vi "GetTestFilterv3.vi"() -> ()   [LabVIEW 2017]
uses:
  <vilib>/httpClient/LabVIEWHTTPClient.lvlib
panel:
  out "result string":string
  out "data":T1
  out "error out":errorcluster
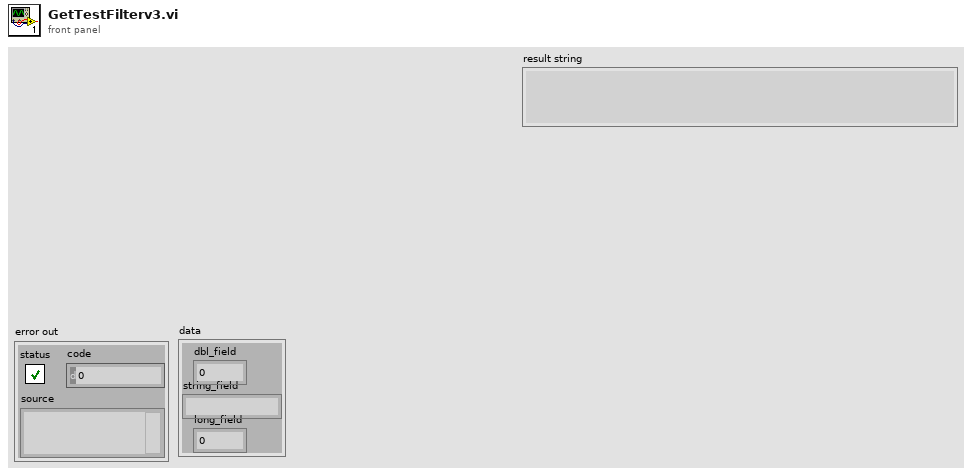
[diagram p1: front panel]
types:
  T1 = cluster{"dbl_field":dbl, "string_field":string, "long_field":i64}
  T2 = typedef "LabVIEWHTTPClient.lvlib/ClientHandle.ctl" = refnum<k1>
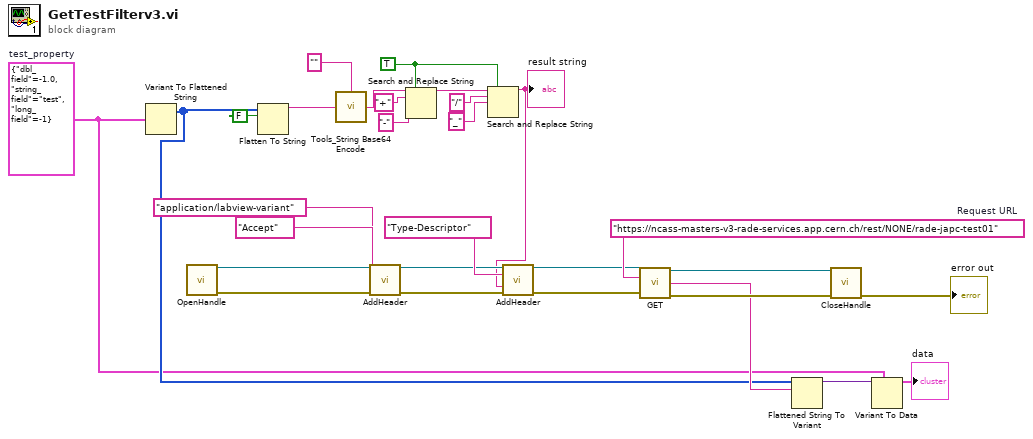
[diagram p0: block diagram]
diagram:
  w1 = T1 {"dbl_field"=-1.0, "string_field"="test", "long_field"=-1}  # test_property
  w7 = TRUE ("replace all? (F)")
  w26 = "https://ncass-masters-v3-rade-services.app.cern.ch/rest/NONE/rade-japc-test01"  # Request URL
  n1 = Variant To Flattened String(Variant=w1) -> (1:w2:i16[])  [unwired: 1 out]
  n2 = call <vilib>:"OpenHandle.vi"() -> ("client handle out"=w20:T2, "error out"=w19:errorcluster)  [unwired: 14 in]
  n3 = Flatten To String(anything=w2, prepend array or string size? (T)=FALSE) -> (data string=w13:string)  [unwired: 2 in, 2 out]
  n4 = call <userlib>:"Tools_String Base64 Encode.vi"("Normal String"=w13, "Line separator (\\n)"="") -> ("Base64 String"=w9:string)
  n5 = call <vilib>:"AddHeader.vi"("client handle"=w20, "header"="Accept", "value"="application/labview-variant", "error in (no error)"=w19) -> ("client handle out"=w18:T2, "error out"=w17:errorcluster)  [unwired: 10 in]
  n6 = Search and Replace String(replace all?=w7, input string=w9, search string="+" ("substring (\"\")"), replace string="-" ("replace string (\"\")")) -> (result string=w8:string)  [unwired: 4 in, 3 out]
  n7 = Search and Replace String(replace all?=w7, input string=w8, search string="/" ("substring (\"\")"), replace string="_" ("replace string (\"\")")) -> (result string=w3:string)  [unwired: 4 in, 3 out]
  "result string" <- w3
  n8 = call <vilib>:"AddHeader.vi"("client handle"=w18, "header"="Type-Descriptor", "value"=w3, "error in (no error)"=w17) -> ("client handle out"=w16:T2, "error out"=w15:errorcluster)  [unwired: 10 in]
  n9 = call <vilib>:"GET.vi"("client handle"=w16, "url"=w26, "error in (no error)"=w15) -> ("client handle out"=w28:T2, "body"=w24:string, "error out"=w25:errorcluster)  [unwired: 9 in, 1 out]
  n10 = Flattened String To Variant(6:w24, 7:w2) -> (3:w23:variant)  [unwired: 1 in, 1 out]
  n11 = call <vilib>:"CloseHandle.vi"("client handle"=w28, "error in (no error)"=w25) -> ("error out"=→"error out":errorcluster)  [unwired: 13 in]
  n12 = Variant To Data(type=w1, Variant=w23) -> (data=→"data":T1)  [unwired: 1 in, 1 out]
